vi "D4xxx Get Values.vi"(8 "error in":errorcluster, 11 "4xxx":refnum<visa-resource-name>) -> (0 "error out":errorcluster, 1 "Frequency":dbl, 2 "Value":dbl, 3 "Session Out":refnum<visa-resource-name>)   [LabVIEW 2009]
doc: "Query set value and set frequency of Datron 4xxx series calibrators."
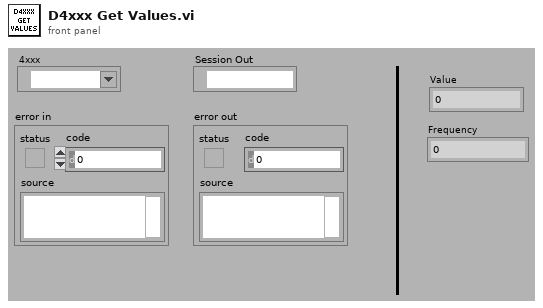
[diagram p1: front panel]
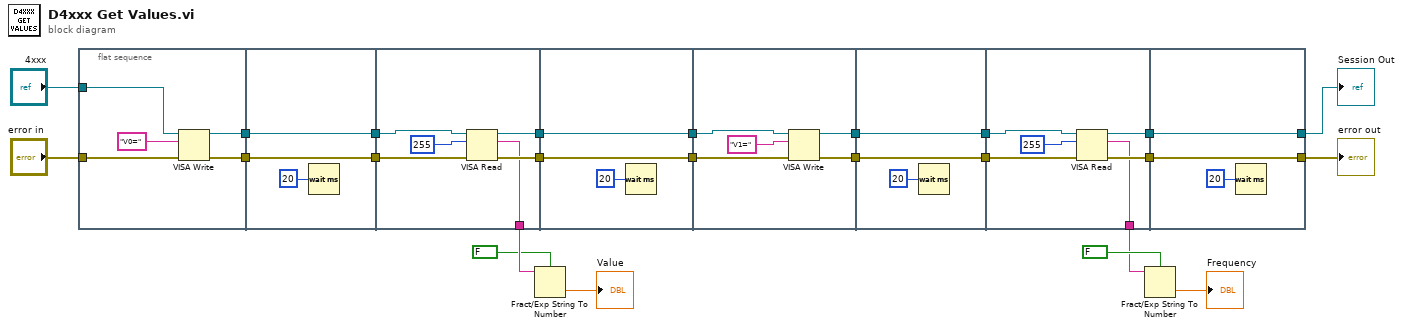
[diagram p0: block diagram]
diagram:
  n1 = flat-sequence {
    tunnel: "4xxx" -> [w28]
    tunnel: "error in" -> [w27]
    tunnel: [w26] -> w22
    tunnel: [w25] -> w21
    tunnel: w22 -> [w31]
    tunnel: w21 -> [w30]
    tunnel: [w31] -> w20
    tunnel: [w30] -> w19
    tunnel: w20 -> [w37]
    tunnel: w19 -> [w36]
    tunnel: [w35] -> w18
    tunnel: [w34] -> w17
    tunnel: [w33] -> w5
    tunnel: w18 -> [w40]
    tunnel: w17 -> [w39]
    tunnel: [w40] -> w16
    tunnel: [w39] -> w15
    tunnel: w16 -> [w45]
    tunnel: w15 -> [w44]
    tunnel: [w43] -> w14
    tunnel: [w42] -> w13
    tunnel: w14 -> [w48]
    tunnel: w13 -> [w47]
    tunnel: [w48] -> w12
    tunnel: [w47] -> w11
    tunnel: w12 -> [w54]
    tunnel: w11 -> [w53]
    tunnel: [w52] -> w10
    tunnel: [w51] -> w9
    tunnel: [w50] -> w2
    tunnel: w10 -> [w57]
    tunnel: w9 -> [w56]
    tunnel: [w57] -> w8
    tunnel: [w56] -> w7
    frame #0 {
      n2 = VISA Write(VISA resource name=w28, write buffer="V0=", error in (no error)=w27) -> (VISA resource name out=w26:refnum<visa-resource-name>, error out=w25:errorcluster)  [unwired: 1 out]
    }
    frame #1 {
      n3 = Wait (ms)(milliseconds to wait=u32 20 ("millisecond multiple")) -> ()  [unwired: 1 out]
    }
    frame #2 {
      n4 = VISA Read(VISA resource name=w37, byte count=u32 255, error in (no error)=w36) -> (VISA resource name out=w35:refnum<visa-resource-name>, read buffer=w33:string, error out=w34:errorcluster)  [unwired: 1 out]
    }
    frame #3 {
      n5 = Wait (ms)(milliseconds to wait=u32 20 ("millisecond multiple")) -> ()  [unwired: 1 out]
    }
    frame #4 {
      n6 = VISA Write(VISA resource name=w45, write buffer="V1=", error in (no error)=w44) -> (VISA resource name out=w43:refnum<visa-resource-name>, error out=w42:errorcluster)  [unwired: 1 out]
    }
    frame #5 {
      n7 = Wait (ms)(milliseconds to wait=u32 20 ("millisecond multiple")) -> ()  [unwired: 1 out]
    }
    frame #6 {
      n8 = VISA Read(VISA resource name=w54, byte count=u32 255, error in (no error)=w53) -> (VISA resource name out=w52:refnum<visa-resource-name>, read buffer=w50:string, error out=w51:errorcluster)  [unwired: 1 out]
    }
    frame #7 {
      n9 = Wait (ms)(milliseconds to wait=u32 20 ("millisecond multiple")) -> ()  [unwired: 1 out]
    }
  }
  n10 = Fract/Exp String To Number(use system decimal point (T)=FALSE, string=w5) -> (number=→"Value":dbl)  [unwired: 2 in, 1 out]
  n11 = Fract/Exp String To Number(use system decimal point (T)=FALSE, string=w2) -> (number=→"Frequency":dbl)  [unwired: 2 in, 1 out]
  "Session Out" <- w8
  "error out" <- w7
